vi "Destroy Broadcast Events.vi"(8 "error in":errorcluster) -> (0 "error out":errorcluster)   [LabVIEW 2026, in "testCoordinator.lvlib"]
doc: "Destroy the broadcast events, even if there is an incoming error.\n\n<b>NOTE</b>: The contents of this VI are automatically generated and modified by the <b>Tools > DQMH Consortium > DQMH</b> utilities. Consider using those utilities instead of making your own modifications to this VI.\n_____\nBased on DQMH Dev Tools: Project Template 7.1.2.1547."
uses:
  testCoordinator.lvlib
panel:
  # "NOTE: The contents of this VI are automatically generated and modified by the Tools > DQMH Consortium > DQMH utilities. Consider using those utilities instead of making your own modifications to this VI."
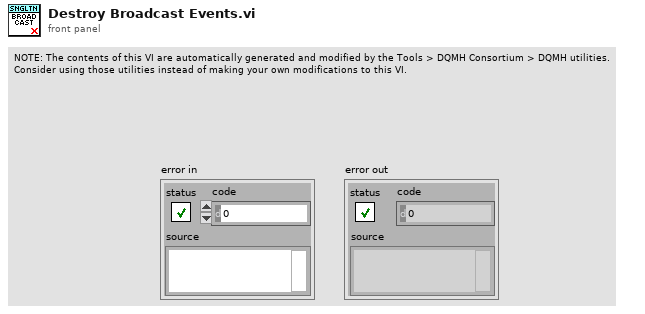
[diagram p1: front panel]
types:
  T1 = typedef "testCoordinator.lvlib/Broadcast Events--cluster.ctl" = cluster{"Module Did Init":refnum<user-event>, "Status Updated":refnum<user-event>, "Error Reported":refnum<user-event>, "Did Something":refnum<user-event>, "Module Did Stop":refnum<user-event>, "Update Module Execution Status":refnum<user-event>, "Broadcast Available Tests":refnum<user-event>, "Refresh Test Procedure Indicator":refnum<user-event>, "Refresh Section Indicator":refnum<user-event>, "Refresh Instruction Indicator":refnum<user-event>, "Broadcast Test Scope":refnum<user-event>, "Broadcast Actual Test Procedure Section":refnum<user-event>}
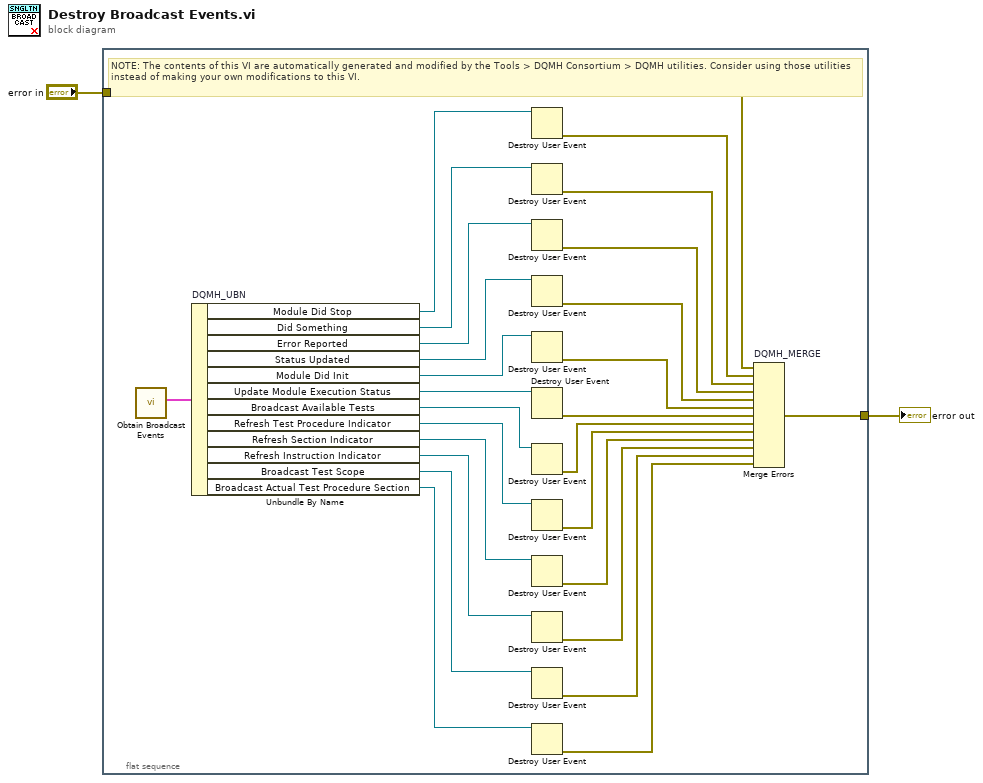
[diagram p0: block diagram]
diagram:
  n1 = flat-sequence {
    tunnel: [w28] -> w2
    tunnel: "error in" -> [w17]
    frame #0 {
      # "NOTE: The contents of this VI are automatically generated and modified by the Tools > DQMH Consortium > DQMH utilities. Consider using those utilities instead of making your own modifications to this VI."
      n2 = call "Obtain Broadcast Events.vi"() -> ("testCoordinator Broadcast Events"=w27:T1)  [unwired: 10 in, 1 out]
      n3 = Unbundle By Name "DQMH_UBN"(w27) -> ("Module Did Stop"=w18:refnum<user-event>, "Did Something"=w21:refnum<user-event>, "Error Reported"=w22:refnum<user-event>, "Status Updated"=w25:refnum<user-event>, "Module Did Init"=w26:refnum<user-event>, "Update Module Execution Status"=w15:refnum<user-event>, "Broadcast Available Tests"=w13:refnum<user-event>, "Refresh Test Procedure Indicator"=w11:refnum<user-event>, "Refresh Section Indicator"=w9:refnum<user-event>, "Refresh Instruction Indicator"=w7:refnum<user-event>, "Broadcast Test Scope"=w5:refnum<user-event>, "Broadcast Actual Test Procedure Section"=w3:refnum<user-event>)
      n4 = Destroy User Event(user event=w18) -> (error out=w19:errorcluster)  [unwired: 1 in]
      n5 = Destroy User Event(user event=w21) -> (error out=w20:errorcluster)  [unwired: 1 in]
      n6 = Destroy User Event(user event=w22) -> (error out=w23:errorcluster)  [unwired: 1 in]
      n7 = Destroy User Event(user event=w25) -> (error out=w24:errorcluster)  [unwired: 1 in]
      n8 = Destroy User Event(user event=w26) -> (error out=w29:errorcluster)  [unwired: 1 in]
      n9 = Destroy User Event(user event=w15) -> (error out=w16:errorcluster)  [unwired: 1 in]
      n10 = Destroy User Event(user event=w13) -> (error out=w14:errorcluster)  [unwired: 1 in]
      n11 = Destroy User Event(user event=w11) -> (error out=w12:errorcluster)  [unwired: 1 in]
      n12 = Destroy User Event(user event=w9) -> (error out=w10:errorcluster)  [unwired: 1 in]
      n13 = Destroy User Event(user event=w7) -> (error out=w8:errorcluster)  [unwired: 1 in]
      n14 = Destroy User Event(user event=w5) -> (error out=w6:errorcluster)  [unwired: 1 in]
      n15 = Destroy User Event(user event=w3) -> (error out=w4:errorcluster)  [unwired: 1 in]
      n16 = Merge Errors "DQMH_MERGE"(w17, w19, w20, w23, w24, w29, w16, w14, w12, w10, w8, w6, w4) -> (w28:errorcluster)
    }
  }
  "error out" <- w2
